vi "HTTP Request.vi"(0 "REST Client in":refnum<class "REST Client.lvclass">, 1 "Request body":string, 2 "Multipart Post data":T1[](array[typedef]), 5 "Method":T2, 9 "Path":string, 11 "error in (no error)":errorcluster, 12 "request specific headers":T3[](array[typedef]), 13 "timeout (0 = Use Default)":i32) -> (3 "Status Code":u16, 4 "REST Client out":refnum<class "REST Client.lvclass">, 6 "Response Headers out":refnum<class "Response Headers.lvclass">, 10 "Response body":string, 14 "Status String":string, 15 "error out":errorcluster)   [LabVIEW 2020, in "REST Client.lvlib" / "REST Client.lvclass"]
uses:
  REST Client.lvclass
  Response Headers/Response Headers.lvclass
  HTTP Header.ctl
  <vilib>/NI/Advanced HTTP Client/Header--Combo Box.ctl
  HTTP Methods.ctl
  <vilib>/httpClient/MultipartData.ctl
  REST Client.lvclass/REST Client.ctl
  http-client/http-client.lvclass
  <vilib>/httpClient/LabVIEWHTTPClient.lvlib
  <vilib>/NI/Advanced HTTP Client/Session.lvclass
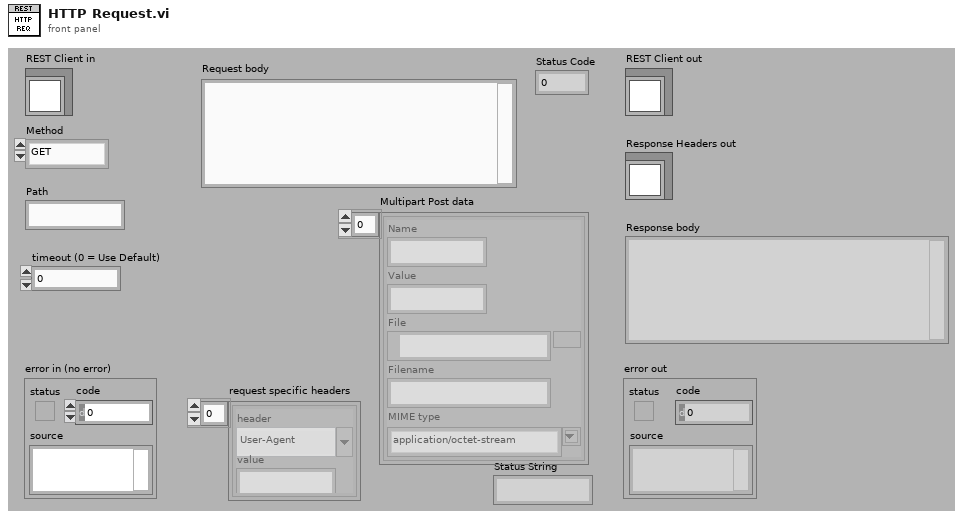
[diagram p1: front panel]
types:
  T1 = typedef "LabVIEWHTTPClient.lvlib/MultipartData.ctl" = cluster{"Name":string, "Value":string, "File":path, "Filename":string, "MIME type":string}
  T2 = typedef "REST Client.lvlib/REST Client.lvclass/HTTP Methods.ctl" = enum16{"GET", "HEAD", "POST", "PUT", "DELETE", "PATCH"}
  T3 = typedef "REST Client.lvlib/REST Client.lvclass/HTTP Header.ctl" = cluster{"header":T4, "value":string}
  T4 = typedef "lib_NI_Advanced HTTP Client.lvlib/Session.lvclass/Header--Combo Box.ctl" = string
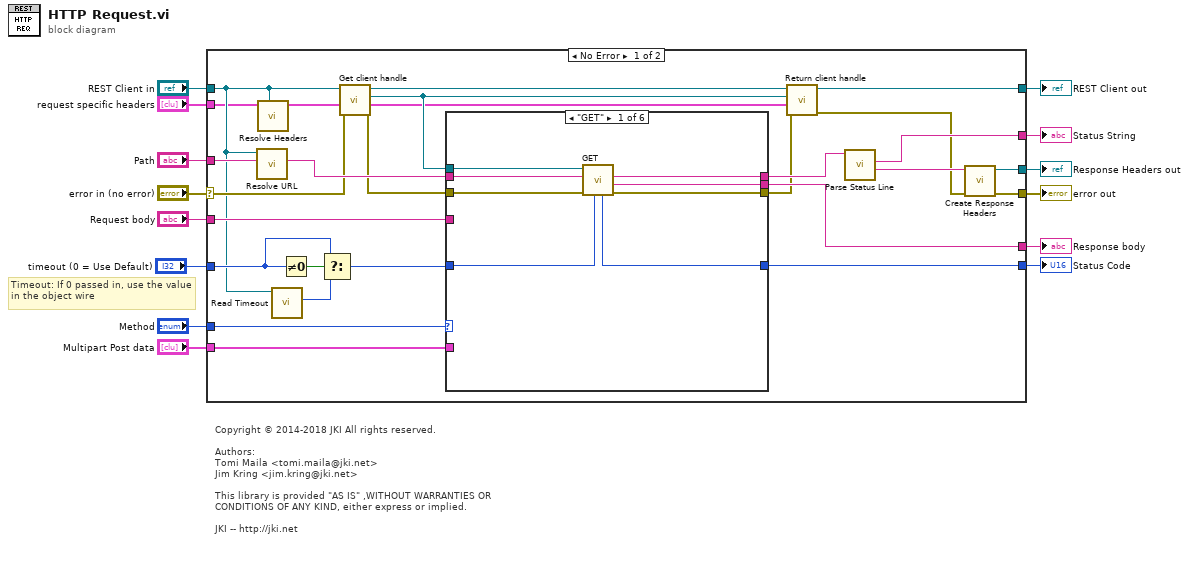
[diagram p0: block diagram]
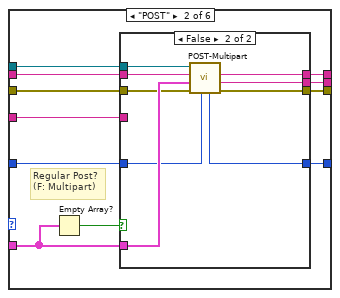
[diagram p2: hidden frame]
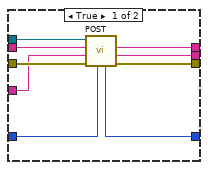
[diagram p3: hidden frame]
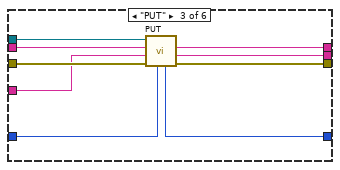
[diagram p4: hidden frame]
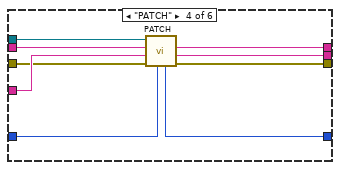
[diagram p5: hidden frame]
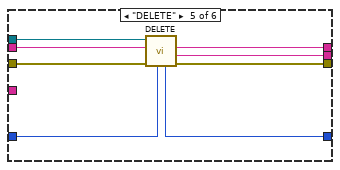
[diagram p6: hidden frame]
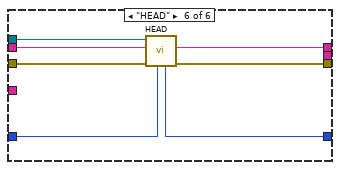
[diagram p7: hidden frame]
diagram:
  # "Timeout: If 0 passed in, use the value in the object wire"
  # "Copyright © 2014-2018 JKI All rights reserved.\n\nAuthors:\nTomi Maila <tomi.maila@jki.net>\nJim Kring <jim.kring@jki.net>\n\nThis library is provided \"AS IS\" ,WITHOUT WARRANTIES OR \nCONDITIONS OF ANY KIND, either express or implied.\n\nJKI -- http://jki.net"
  n1 = case shown="No Error" "error in (no error)" {
    selector: "error in (no error)" -> [w22 w113]
    tunnel: [w18 w113] -> w1
    tunnel: [w17 w112] -> w12
    tunnel: "REST Client in" -> [w21 w112]
    tunnel: "Method" -> [w37 _]
    tunnel: "Path" -> [w36 _]
    tunnel: "Request body" -> [w28 _]
    tunnel: [w25 _] -> w9
    tunnel: [w33 _] -> w4
    tunnel: [w34 _] -> w8
    tunnel: "request specific headers" -> [w20 _]
    tunnel: [w15 _] -> w5
    tunnel: "Multipart Post data" -> [w32 _]
    tunnel: "timeout (0 = Use Default)" -> [w30 _]
    frame No Error {
      n2 = call "Resolve URL.vi"("Path"=w36, "REST Client in"=w21) -> ("Resolved URL"=w35:string)  [unwired: 9 in]
      n3 = call "Resolve Headers.vi"("REST Client in"=w21, "headers in"=w20) -> ("headers out"=w19:T3[])  [unwired: 9 in]
      n4 = call-dynamic "Read Timeout.vi"("REST Client in"=w21) -> ("Timeout"=w26:i32)  [unwired: 8 in, 2 out]
      n5 = Not Equal To 0?(x=w30) -> (x != 0?=w31:bool)
      n6 = Select(t=w30, s=w31, f=w26) -> (s? t:f=w29:i32)
      n7 = call "Get client handle.vi"("error in (no error)"=w22, "headers"=w19, "REST Client in"=w21) -> ("error out"=w27:errorcluster, "headers out"=w38:T3[], "http-client"=w39:refnum<class "http-client.lvclass">, "REST Client out"=w40:refnum<class "REST Client.lvclass">)  [unwired: 5 in]
      n8 = case shown="\"GET\"" w37 {
        tunnel: w35 -> [w48 w60 w80 w96 w103 w111]
        tunnel: w29 -> [w43 w59 w83 w90 w98 w107]
        tunnel: w27 -> [w44 w58 w82 w94 w99 w110]
        tunnel: [w47 w57 w86 w91 w102 w109] -> w41
        tunnel: [w46 w56 w85 w92 w101 _] -> w34
        tunnel: [w45 w55 w84 w93 w100 w108] -> w23
        tunnel: w39 -> [w49 w54 w87 w89 w104 w106]
        tunnel: w32 -> [_ w51 _ _ _ _]
        tunnel: w28 -> [_ w52 w81 w95 _ _]
        tunnel: [w42 w50 w79 w88 w97 w105] -> w15
        frame "GET" {
          n9 = call "GET.vi"("timeout"=w43, "error in"=w44, "url"=w48, "http-client in"=w49) -> ("error out"=w45:errorcluster, "body"=w46:string, "headers"=w47:string, "status code"=w42:u16)  [unwired: 3 in, 1 out]
        }
        frame "POST" {
          # "Regular Post?\n(F: Multipart)"
          n10 = Empty Array?(array=w51) -> (empty?=w53:bool)
          n11 = case shown="False" w53 {
            tunnel: w60 -> [w66 w77]
            tunnel: w59 -> [w64 w71]
            tunnel: w58 -> [w68 w75]
            tunnel: [w63 w72] -> w57
            tunnel: [w62 w73] -> w56
            tunnel: [w67 w74] -> w55
            tunnel: w54 -> [w69 w78]
            tunnel: w52 -> [w65 _]
            tunnel: w51 -> [_ w76]
            tunnel: [w61 w70] -> w50
            frame True {
              n12 = call "POST.vi"("timeout"=w64, "error in"=w68, "buffer"=w65, "url"=w66, "http-client in"=w69) -> ("error out"=w67:errorcluster, "body"=w62:string, "headers"=w63:string, "status code"=w61:u16)  [unwired: 2 in, 1 out]
            }
            frame False {
              n13 = call "POST-Multipart.vi"("timeout"=w71, "error in"=w75, "Multipart Post data"=w76, "url"=w77, "http-client in"=w78) -> ("error out"=w74:errorcluster, "body"=w73:string, "headers"=w72:string, "status code"=w70:u16)  [unwired: 2 in, 1 out]
            }
          }
        }
        frame "PUT" {
          n14 = call "PUT.vi"("timeout"=w83, "error in"=w82, "buffer"=w81, "url"=w80, "http-client in"=w87) -> ("error out"=w84:errorcluster, "body"=w85:string, "headers"=w86:string, "status code"=w79:u16)  [unwired: 2 in, 1 out]
        }
        frame "PATCH" {
          n15 = call "PATCH.vi"("timeout"=w90, "error in"=w94, "buffer"=w95, "url"=w96, "http-client in"=w89) -> ("error out"=w93:errorcluster, "body"=w92:string, "headers"=w91:string, "status code"=w88:u16)  [unwired: 2 in, 1 out]
        }
        frame "DELETE" {
          n16 = call "DELETE.vi"("timeout"=w98, "error in"=w99, "url"=w103, "http-client in"=w104) -> ("error out"=w100:errorcluster, "body"=w101:string, "headers"=w102:string, "status code"=w97:u16)  [unwired: 3 in, 1 out]
        }
        frame "HEAD" {
          n17 = call "HEAD.vi"("timeout"=w107, "error in"=w110, "url"=w111, "http-client in"=w106) -> ("error out"=w108:errorcluster, "headers"=w109:string, "status code"=w105:u16)  [unwired: 4 in, 1 out]
        }
      }
      n18 = call "Return client handle.vi"("error in (no error)"=w23, "headers"=w38, "http-client"=w39, "REST Client in"=w40) -> ("error out"=w16:errorcluster, "REST Client out"=w17:refnum<class "REST Client.lvclass">)  [unwired: 6 in]
      n19 = call "Parse Status Line.vi"("Headers w/ status line"=w41) -> ("HTTP Headers"=w24:string, "Status String"=w25:string)  [unwired: 6 in, 3 out]
      n20 = call "Create Response Headers.vi"("error in (no error)"=w16, "Response Headers"=w24) -> ("error out"=w18:errorcluster, "Response Headers out"=w33:refnum<class "Response Headers.lvclass">)  [unwired: 8 in]
    }
    frame Error {
    }
  }
  "error out" <- w1
  "REST Client out" <- w12
  "Status Code" <- w5
  "Status String" <- w9
  "Response Headers out" <- w4
  "Response body" <- w8
